vi "SetGPIOMode.vi"(7 "Channel":u8, 8 "error in (no error)":errorcluster, 9 "Op Mode":T2=3 items=["M5_8SERVOS2_MODE_INPUT  ", "M5_8SERVOS2_MODE_OUTPUT ", "M5_8SERVOS2_MODE_ADC    ", "M5_8SERVOS2_MODE_SERVO  ", "M5_8SERVOS2_MODE_RGB    ", "M5_8SERVOS2_MODE_PWM    "], 10 "Registers":T1 items=["UNIT_8SERVOS2_REG_MODE_START"=0, "UNIT_8SERVOS2_REG_INPUT_PULL_START"=16, "UNIT_8SERVOS2_REG_INPUT_STATUS_START"=32, "UNIT_8SERVOS2_REG_OUTPUT_STATUS_START"=48, "UNIT_8SERVOS2_REG_ADC_START"=64, "UNIT_8SERVOS2_REG_SERVO_START"=80, "UNIT_8SERVOS2_REG_RGB_CONF_START"=96, "UNIT_8SERVOS2_REG_PWM_DUTY_START"=112, "UNIT_8SERVOS2_REG_RGB_BUFFER_START"=128, "UNIT_8SERVOS2_REG_TIM_FREQ_START"=208, "UNIT_8SERVOS2_REG_UID_START"=224, "UNIT_8SERVOS2_REG_UID_END"=235, "UNIT_8SERVOS2_REG_SYS_ANALOG_START"=240, "UNIT_8SERVOS2_REG_ADDR_OFFSET"=248, "UNIT_8SERVOS2_REG_I2C_ADDR_REFRESH"=252, "UNIT_8SERVOS2_REG_VERSION"=254, "UNIT_8SERVOS2_REG_I2C_ADDR"=255], 11 "M5Stack I2C 8Ch Servo in":refnum<class "M5Stack I2C 8Ch Servo.lvclass">) -> (0 "error out":errorcluster, 3 "M5Stack I2C 8Ch Servo out":refnum<class "M5Stack I2C 8Ch Servo.lvclass">)   [LabVIEW 2020, in "CTI-Peripheral.lvlib" / "M5Stack I2C 8Ch Servo.lvclass"]
uses:
  M5Stack I2C 8Ch Servo.lvclass
  Private/GPIOOperationModes.ctl
  Private/registers.ctl
  M5Stack I2C 8Ch Servo.lvclass/M5Stack I2C 8Ch Servo.ctl
  CTI/I2C Connection/I2C Connection.lvclass/I2C Connection.ctl
  CTI/Session/I2C Write Data.vi
  CTI/I2C Connection/I2C Connection.lvclass
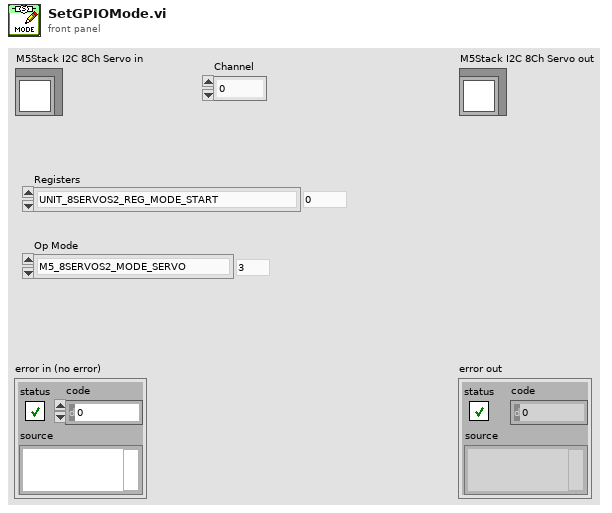
[diagram p1: front panel]
types:
  T1 = typedef "CTI-Peripheral.lvlib/M5Stack I2C 8Ch Servo.lvclass/registers.ctl" = u8
  T2 = typedef "CTI-Peripheral.lvlib/M5Stack I2C 8Ch Servo.lvclass/GPIOOperationModes.ctl" = u16
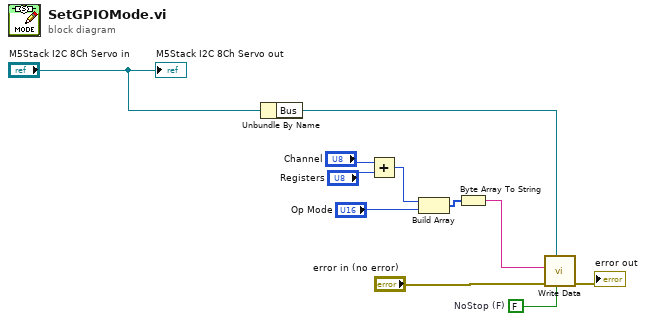
[diagram p0: block diagram]
diagram:
  w11 = FALSE  # NoStop (F)
  n1 = Unbundle By Name("M5Stack I2C 8Ch Servo in") -> ("Bus"=w5:refnum<class "I2C Connection.lvclass">)
  n2 = Add(x="Channel", y="Registers") -> (x+y=w3:T1)
  n3 = Build Array(w3, "Op Mode") -> (w9:T2[])
  n4 = Byte Array To String(unsigned byte array=w9) -> (string=w8:string)
  n5 = call "Write Data.vi"("NoStop (F)"=w11, "I2C Connection"=w5, "error in (no error)"="error in (no error)", "Data"=w8) -> ("error out"=→"error out":errorcluster)  [unwired: 7 in]
  "M5Stack I2C 8Ch Servo out" <- "M5Stack I2C 8Ch Servo in"
